vi "PathPlanner_PathFinder_InitializeWorkerThread.vi"   [LabVIEW 2019, in "PathPlanner24.lvlib"]
doc: "Internal function. Not to be used by end users."
uses:
  PathPlanner24.lvlib
  PathPlanner_PathFinder_Globals.vi
  PathPlanner_PathFinder_WorkerThreadALT.vi
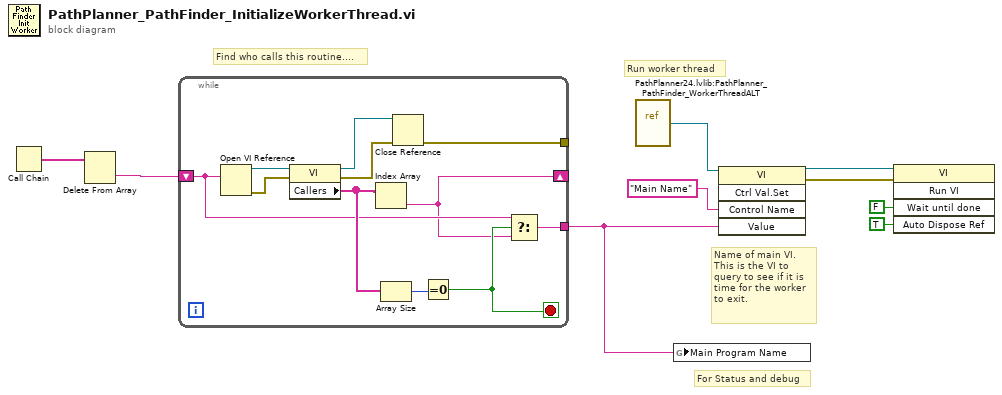
[diagram p0: block diagram]
diagram:
  # "For Status and debug"
  # "Find who calls this routine...."
  # "Name of main VI.\nThis is the VI to \nquery to see if it is\ntime for the worker\nto exit."
  # "Run worker thread"
  n1 = Call Chain() -> (call chain=w3:string[])
  n2 = Delete From Array(array=w3) -> (deleted portion=w2:string)  [unwired: 2 in, 1 out]
  n3 = while {
    shift-right: [w14] -> _
    shift-left: w2 -> [w15]
    tunnel: [w13] -> w4
    tunnel: [w10] -> _
    stop <- w16 stop-if-true
    n4 = Open VI Reference(vi path=w15) -> (vi reference=w20:refnum<vi>, error out=w12:errorcluster)  [unwired: 5 in]
    n5 = property class="VI"(reference=w20, error in=w12) -> (reference out=w19:refnum<vi>, error out=w11:errorcluster, "Callers"=w18:string[])
    n6 = Index Array(array=w18) -> (element=w14:string)  [unwired: 1 in]
    n7 = Array Size(array=w18) -> (size(s)=w17:i32)
    n8 = Close Reference(reference=w19, error in (no error)=w11) -> (error out=w10:errorcluster)
    n9 = Equal To 0?(x=w17) -> (x = 0?=w16:bool)
    n10 = Select(t=w15, s=w16, f=w14) -> (s? t:f=w13:string)
  }
  n11 = vi-ref "PathPlanner24.lvlib:PathPlanner_PathFinder_WorkerThreadALT.vi"() -> (w1:refnum<vi>)
  n12 = global write "PathPlanner_PathFinder_Globals.vi" "Main Program Name"(w4) -> ()
  n13 = invoke class="VI" method="Ctrl Val.Set"(reference=w1, "Control Name"="Main Name", "Value"=w4) -> (reference out=w8:refnum<vi>, error out=w7:errorcluster)  [unwired: 2 in, 3 out]
  n14 = invoke class="VI" method="Run VI"(reference=w8, error in=w7, "Wait until done"=FALSE ("Wait Until Done"), "Auto Dispose Ref"=TRUE ("Auto Dispose Reference")) -> ()  [unwired: 1 in, 5 out]
